vi "Close.vi"(8 "error in (no error)":errorcluster, 11 "DAQNavi_AI in":refnum<class "DAQNavi_AI.lvclass">) -> (0 "error out":errorcluster, 3 "DAQNavi_AI out":refnum<class "DAQNavi_AI.lvclass">)   [LabVIEW 2021, in "DAQNavi_AI.lvclass"]
uses:
  DAQNavi_AI.lvclass
  DAQNavi_AI.lvclass/DAQNavi_AI.ctl
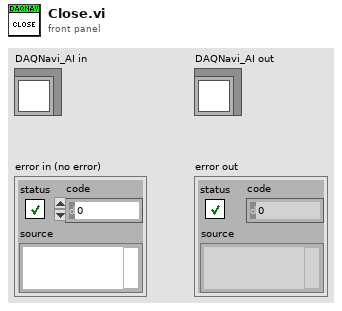
[diagram p1: front panel]
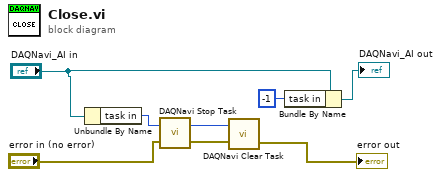
[diagram p0: block diagram]
diagram:
  n1 = Unbundle By Name("DAQNavi_AI in") -> ("task in"=w6:i32)
  n2 = call <userlib>:"DAQNavi Stop Task.vi"("error in (no error)"="error in (no error)", "task in"=w6) -> ("error out"=w7:errorcluster, "task out"=w8:i32)
  n3 = call <userlib>:"DAQNavi Clear Task.vi"("error in (no error)"=w7, "task in"=w8) -> ("error out"=→"error out":errorcluster)  [unwired: 1 in]
  n4 = Bundle By Name(cluster="DAQNavi_AI in", "task in"=-1) -> (→"DAQNavi_AI out":refnum<class "DAQNavi_AI.lvclass">)
